vi "Build VIHelpeks Project.vi"(7 "Show Progress Window (T)":bool=TRUE, 8 "error in":errorcluster, 9 "Generate CHM (T)":bool=TRUE, 10 "Generate HHP (T)":bool=TRUE, 11 "VIHelpeks Project File":path) -> (0 "error out":errorcluster, 1 "Errors":i32, 2 "Paths":T1, 3 "dup VIHelpeks Project File":path)   [LabVIEW 2014, in "VIHelpeksAPI.lvlib"]
doc: "The VI builds help files based on a <b>VIHelpeks Project File</b>. The project file must be created and configured beforehand using the VI Helpeks UI (the help project manager). Information regarding the compiled project can be found in the files returned by the <b>Paths</b> indicator.\n\nThe VI generates a set of HTML files. In addition, if enabled, it generates project files for Microsoft HTML Help Workshop (.HHP and related files). Afterwards, if enabled, it compiles a final .CHM file based on the created (or already existing) .HHP and HTML files.\n\n<b>NOTICE:</b> In order to generate a CHM file, it is required to have Microsoft HTML Help Workshop installed on your computer. You can download it on the Microsoft website for free: <b>http://msdn.microsoft.com/en-us/library/ms669985.aspx</b>.\n\nThe <b>Example VI</b> demonstrating the use of VIHelpeks API can be opened using the \"Tools >> VI Helpeks >> Help and Support\" menu. Alternatively, you can launch the <b>NI Example Finder</b> and search for \"VI Helpeks\", or find it within the <b><labview>\\Examples\\VI Helpeks</b> folder.\n\n::: VI Helpeks :::\nCopyright (c) 2000-2026 Konstantin Shifershteyn. All rights reserved."
uses:
  VIHelpeksAPI.lvlib
  <vilib>/Utility/error.llb/DialogType.ctl
panel:
  in  "Show Window":bool
  out "VIHelpeks message":string
  # "VI Helpeks\nCopyright (c) 2012-2026 Konstantin Shifershteyn"
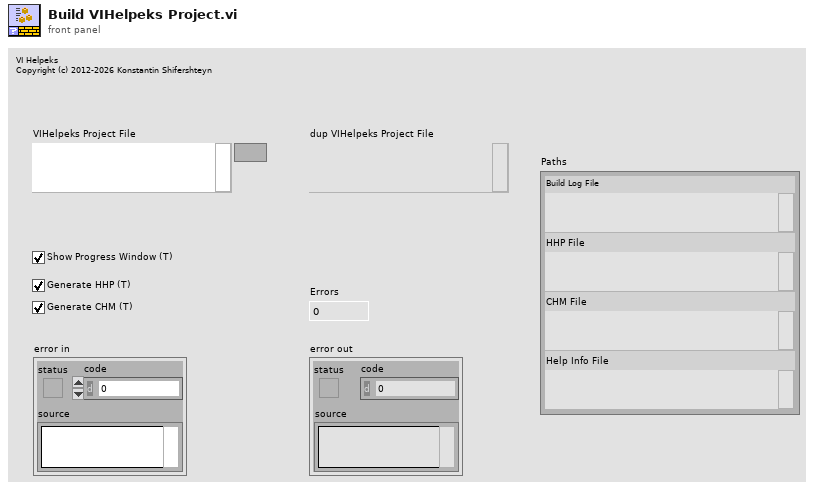
[diagram p1: front panel]
types:
  T1 = cluster{"Build Log File":path, "HHP File":path, "CHM File":path, "Help Info File":path}
  T2 = cluster{"HTML Build Log":path, "HHP File":path, "CHM File":path, "CHM Info File":path}
  T3 = cluster{"queue out":refnum<queue>, "queue out":refnum<queue>}
  T4 = cluster{"Msg":string, "Data":string, "error":errorcluster}
  T5 = enum32{"Bad", "Idle", "Run top level", "Running"}
  T6 = typedef "DialogType.ctl" = u16
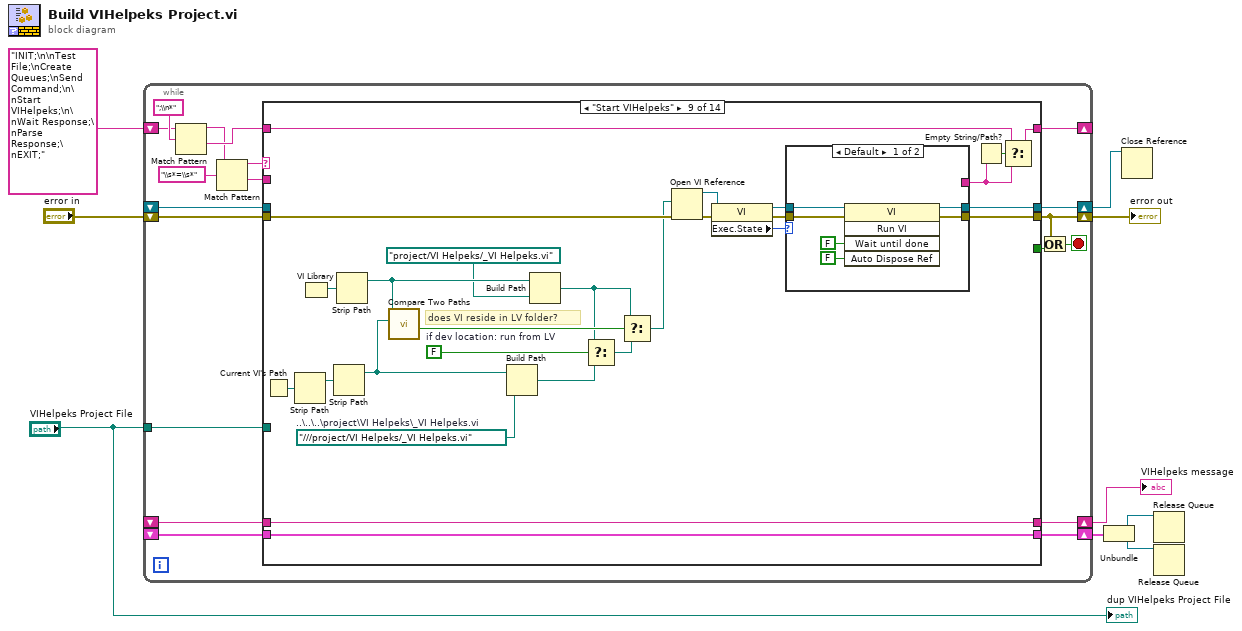
[diagram p0: block diagram]
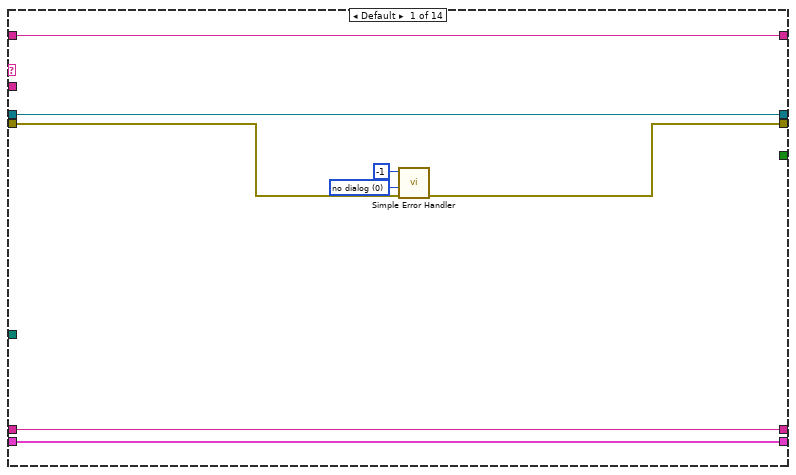
[diagram p2: hidden frame]
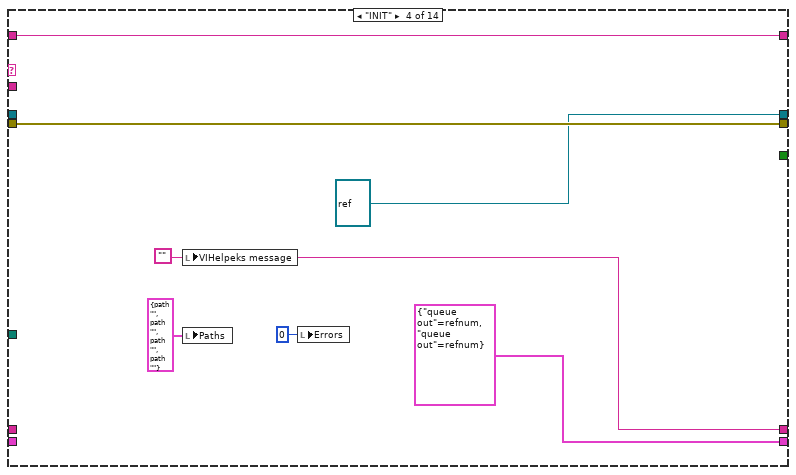
[diagram p5: hidden frame]
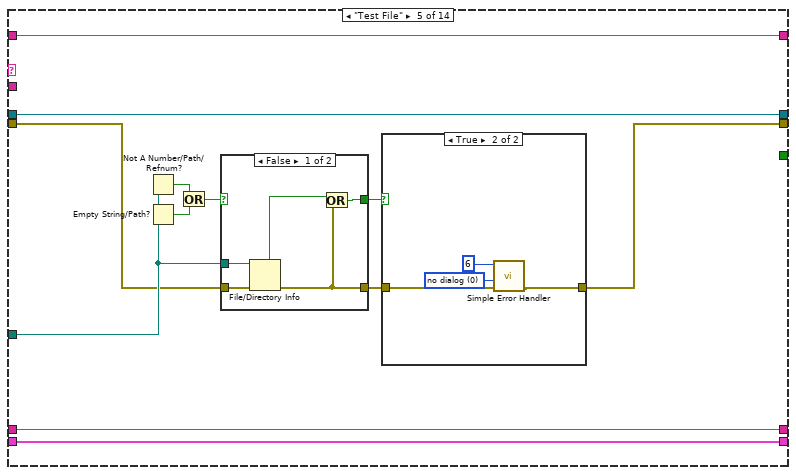
[diagram p6: hidden frame]
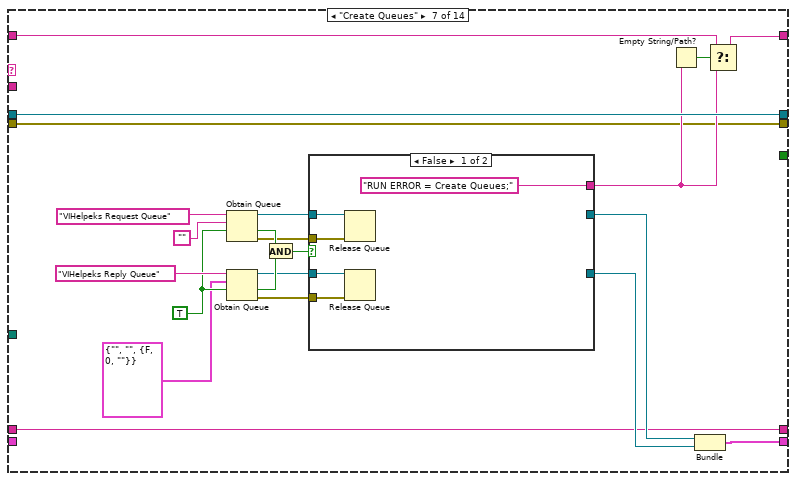
[diagram p10: hidden frame]
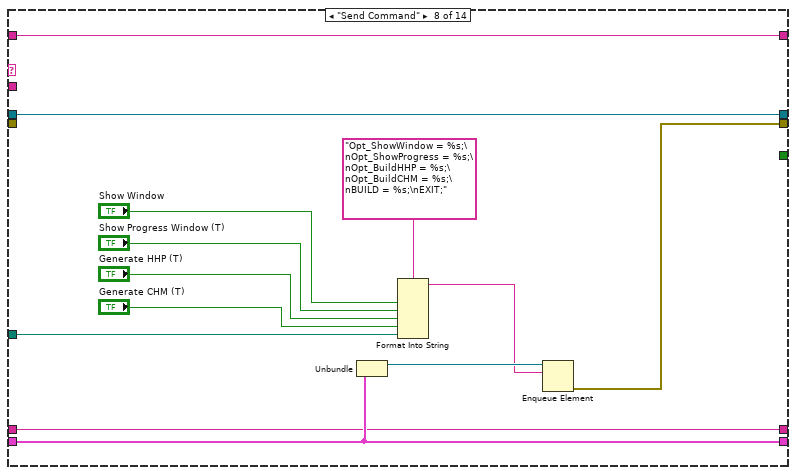
[diagram p12: hidden frame]
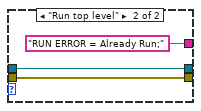
[diagram p13: hidden frame]
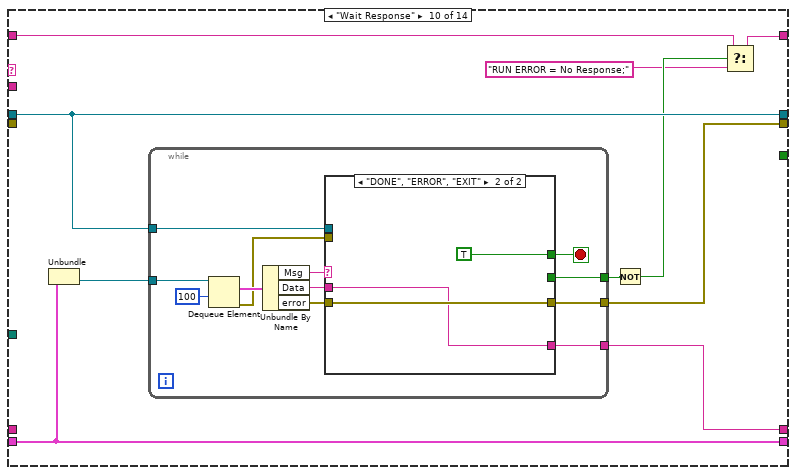
[diagram p14: hidden frame]
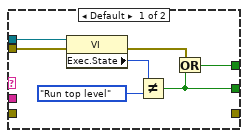
[diagram p15: hidden frame]
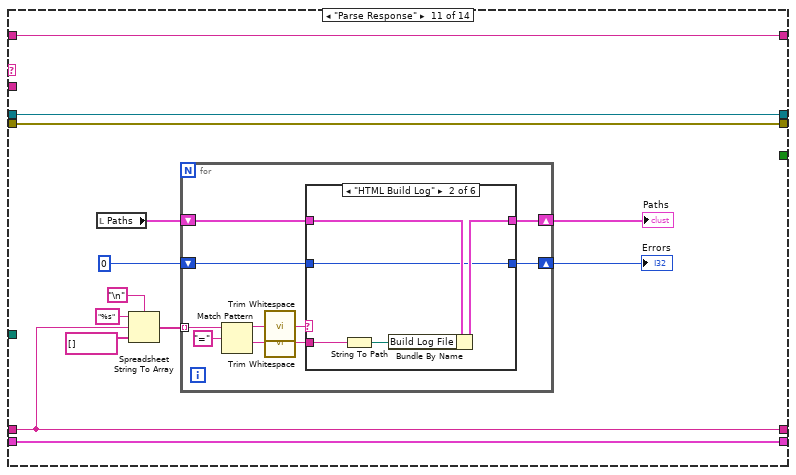
[diagram p16: hidden frame]
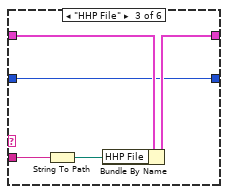
[diagram p18: hidden frame]
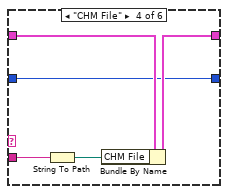
[diagram p19: hidden frame]
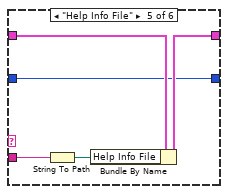
[diagram p20: hidden frame]
diagram:
  n1 = while {
    shift-right: [w26] -> _
    shift-left: "INIT;\n\nTest File;\nCreate Queues;\nSend Command;\n\nStart VIHelpeks;\n\nWait Response;\nParse Response;\nEXIT;" -> [w27]
    shift-right: [w19] -> w7
    shift-left: "error in" -> [w24]
    tunnel: "VIHelpeks Project File" -> [w22]
    shift-right: [w21] -> w6
    shift-left: _ -> [w20]
    shift-right: [w17] -> w5
    shift-left: _ -> [w16]
    shift-right: [w11] -> w2
    shift-left: _ -> [w10]
    stop <- w23 stop-if-true
    n2 = Match Pattern(string=w27, regular expression=";\\n*") -> (before substring=w15:string, after substring=w25:string)  [unwired: 1 in, 2 out]
    n3 = Match Pattern(string=w15, regular expression="\\s*=\\s*") -> (before substring=w13:string, after substring=w12:string)  [unwired: 1 in, 2 out]
    n4 = case shown="\"Start VIHelpeks\"" w13 {
      tunnel: [w36 w41 w46 w52 w57 w82 w87 w118 w140 w165 w205 w245 w262 w274] -> w26
      tunnel: w25 -> [w36 w41 w46 w52 w57 w82 w88 w118 w141 w161 w205 w245 w262 w274]
      tunnel: w24 -> [w35 w38 w43 w53 w60 w79 w84 _ w146 _ w203 w242 w258 w270]
      tunnel: [w34 w38 w43 w53 w59 w79 w84 w119 w145 w163 w203 w242 w257 w270] -> w19
      tunnel: w22 -> [_ _ _ _ w63 _ _ w121 _ _ _ _ _ _]
      tunnel: [w32 w40 w45 refnum<vi> refnum ("vi reference") w56 w81 w104 w124 w144 w168 w202 w244 w261 w273] -> w21
      tunnel: w20 -> [w32 w40 w45 _ w56 w81 w104 w124 _ w168 w202 w244 w261 w273]
      tunnel: [_ _ _ _ _ _ _ _ _ _ _ _ TRUE TRUE] -> w18
      tunnel: [w31 w39 w44 T3 {"queue out"=refnum, "queue out"=refnum} ("output cluster") w55 w80 w90 w123 w143 w170 w204 w243 w259 w271] -> w17
      tunnel: w16 -> [w31 w39 w44 _ w55 w80 _ w123 w143 w170 w204 w243 w259 w271]
      tunnel: w12 -> [_ _ _ _ _ _ _ _ _ _ _ _ w255 _]
      tunnel: [w29 w37 w42 w49 w54 w78 w83 w112 w128 w162 w200 w241 w246 w269] -> w11
      tunnel: w10 -> [w29 w37 w42 _ w54 w78 w83 w112 w128 _ w200 w241 w246 w269]
      frame Default {
        w30 = T6 0 items=["no dialog", "OK message", "continue or stop message", "OK message + warnings", "continue/stop + warnings"] ("type of dialog (OK msg:1)")
        n5 = call <vilib>:"Simple Error Handler.vi"("error code (no error:0)"=-1, "type of dialog (OK msg:1)"=w30, "error in (no error)"=w35) -> ("error out"=w34:errorcluster)  [unwired: 2 in, 4 out]
      }
      frame "" {
      }
      frame "------------------- 1" {
      }
      frame "INIT" {
        w49 = ""
        n6 = local write "VIHelpeks message"(w49) -> ()
        n7 = local write "Paths"(T2 {"HTML Build Log"=path "", "HHP File"=path "", "CHM File"=path "", "CHM Info File"=path ""} ("Paths")) -> ()
        n8 = local write "Errors"(0 ("Errors")) -> ()
      }
      frame "Test File" {
        n9 = Not A Number/Path/Refnum?(number/path/refnum=w63) -> (NaN/Path/Refnum?=w65:bool)
        n10 = Empty String/Path?(string/path=w63) -> (empty?=w64:bool)
        n11 = Or(x=w65, y=w64) -> (x .or. y?=w62:bool)
        n12 = case shown="False" w62 {
          selector: w62 -> [_ w77]
          tunnel: w63 -> [w75 _]
          tunnel: [w74 w77] -> w61
          tunnel: w60 -> [w72 w76]
          tunnel: [w71 w76] -> w58
          frame False {
            n13 = File/Directory Info(path=w75, error in=w72) -> (directory=w73:bool, error out=w71:errorcluster)  [unwired: 5 out]
            n14 = Or(x=w73, y=w71) -> (x .or. y?=w74:bool)
          }
          frame True {
          }
        }
        n15 = case shown="True" w61 {
          tunnel: [w66 w69] -> w59
          tunnel: w58 -> [w66 w70]
          frame False {
          }
          frame True {
            w67 = T6 0 items=["no dialog", "OK message", "continue or stop message", "OK message + warnings", "continue/stop + warnings"] ("type of dialog (OK msg:1)")
            n16 = call <vilib>:"Simple Error Handler.vi"("error code (no error:0)"=6, "type of dialog (OK msg:1)"=w67, "error in (no error)"=w70) -> ("error out"=w69:errorcluster)  [unwired: 2 in, 4 out]
          }
        }
      }
      frame "------------------- 2" {
      }
      frame "Create Queues" {
        w100 = TRUE
        n17 = Obtain Queue(name (unnamed)="VIHelpeks Request Queue", element data type="", create if not found? (T)=w100) -> (queue out=w96:refnum<queue>, created new?=w99:bool, error out=w94:errorcluster)  [unwired: 2 in]
        n18 = Obtain Queue(name (unnamed)="VIHelpeks Reply Queue", element data type=T4 {"Msg"="", "Data"="", "error"={"status"=FALSE, "code"=0, "source"=""}}, create if not found? (T)=w100) -> (queue out=w95:refnum<queue>, created new?=w98:bool, error out=w93:errorcluster)  [unwired: 2 in]
        n19 = And(x=w99, y=w98) -> (x .and. y?=w97:bool)
        n20 = case shown="False" w97 {
          tunnel: [_ w111] -> w92
          tunnel: w96 -> [w108 w111]
          tunnel: [_ w110] -> w91
          tunnel: w95 -> [w109 w110]
          tunnel: w94 -> [w107 _]
          tunnel: w93 -> [w106 _]
          tunnel: ["RUN ERROR = Create Queues;" _] -> w86
          frame False {
            n21 = Release Queue(queue=w108, error in (no error)=w107) -> ()  [unwired: 1 in, 3 out]
            n22 = Release Queue(queue=w109, error in (no error)=w106) -> ()  [unwired: 1 in, 3 out]
          }
          frame True {
          }
        }
        n23 = Empty String/Path?(string/path=w86) -> (empty?=w85:bool)
        n24 = Bundle("queue out"=w92, "queue out"=w91) -> (w90:T3)  [unwired: 1 in]
        n25 = Select(t=w88, s=w85, f=w86) -> (s? t:f=w87:string)
      }
      frame "Send Command" {
        n26 = Unbundle(w123) -> ("queue out"=w122:refnum<queue>)  [unwired: 1 out]
        n27 = Format Into String(format string="Opt_ShowWindow = %s;\nOpt_ShowProgress = %s;\nOpt_BuildHHP = %s;\nOpt_BuildCHM = %s;\nBUILD = %s;\nEXIT;", "Show Window", "Show Progress Window (T)", "Generate HHP (T)", "Generate CHM (T)", w121) -> (resulting string=w120:string)  [unwired: 2 in, 1 out]
        n28 = Enqueue Element(queue=w122, element=w120) -> (error out=w119:errorcluster)  [unwired: 2 in, 2 out]
      }
      frame "Start VIHelpeks" {
        w130 = FALSE  # if dev location: run from LV
        w134 = path "../../../project/VI Helpeks/_VI Helpeks.vi"  # ..\..\..\project\VI Helpeks\_VI Helpeks.vi
        # "does VI reside in LV folder?"
        n29 = Current VI's Path() -> (path=w127:path)
        n30 = Strip Path(path=w127) -> (stripped path=w126:path)  [unwired: 1 out]
        n31 = VI Library() -> (path=w138:path)
        n32 = Strip Path(path=w126) -> (stripped path=w125:path)  [unwired: 1 out]
        n33 = Strip Path(path=w138) -> (stripped path=w137:path)  [unwired: 1 out]
        n34 = call <vilib>:"Compare Two Paths.vi"("Path 2"=w125, "Path 1"=w137) -> ("Path 2 Relative to Path 1?"=w135:bool)  [unwired: 6 in, 3 out]
        n35 = Build Path(base path=w125, name or relative path=w134) -> (appended path=w131:path)
        n36 = Build Path(base path=w137, name or relative path=path "project/VI Helpeks/_VI Helpeks.vi") -> (appended path=w133:path)
        n37 = Select(t=w133, s=w130, f=w131) -> (s? t:f=w132:path)
        n38 = Select(t=w133, s=w135, f=w132) -> (s? t:f=w129:path)
        n39 = Open VI Reference(vi path=w129, error in (no error)=w146) -> (vi reference=w148:refnum<vi>, error out=w147:errorcluster)  [unwired: 4 in]
        n40 = property class="VI"(reference=w148, error in=w147) -> (reference out=w151:refnum<vi>, error out=w150:errorcluster, "Exec.State"=w149:T5)
        n41 = case shown="Default" w149 {
          tunnel: [w153 w160] -> w145
          tunnel: w150 -> [w155 w160]
          tunnel: w151 -> [w154 w159]
          tunnel: [w152 w159] -> w144
          tunnel: [_ "RUN ERROR = Already Run;"] -> w139
          frame Default {
            n42 = invoke class="VI" method="Run VI"(reference=w154, error in=w155, "Wait until done"=FALSE ("Wait Until Done"), "Auto Dispose Ref"=FALSE ("Auto Dispose Reference")) -> (reference out=w152:refnum<vi>, error out=w153:errorcluster)  [unwired: 1 in, 3 out]
          }
          frame "Run top level" {
          }
        }
        n43 = Empty String/Path?(string/path=w139) -> (empty?=w142:bool)
        n44 = Select(t=w141, s=w142, f=w139) -> (s? t:f=w140:string)
      }
      frame "Wait Response" {
        n45 = Unbundle(w170) -> ("queue out"=w169:refnum<queue>)  [unwired: 1 out]
        n46 = while {
          tunnel: w169 -> [w182]
          tunnel: w168 -> [w177]
          tunnel: [w173] -> w167
          tunnel: [w172] -> w163
          tunnel: [w171] -> w162
          stop <- w176 stop-if-true
          n47 = Dequeue Element(queue=w182, timeout in ms (-1)=100) -> (element=w180:T4, error out=w175:errorcluster)  [unwired: 1 in, 2 out]
          n48 = Unbundle By Name(w180) -> ("Msg"=w179:string, "Data"=w174:string, "error"=w178:errorcluster)
          n49 = case shown="\"DONE\", \"ERROR\", \"EXIT\"" w179 {
            tunnel: w178 -> [_ w191]
            tunnel: w177 -> [w186 _]
            tunnel: [w185 TRUE] -> w176
            tunnel: w175 -> [w184 _]
            tunnel: w174 -> [_ w190]
            tunnel: [w183 _] -> w173
            tunnel: [_ w191] -> w172
            tunnel: [_ w190] -> w171
            frame Default {
              n50 = property class="VI"(reference=w186, error in=w184) -> (error out=w187:errorcluster, "Exec.State"=w189:T5)  [unwired: 1 out]
              n51 = Not Equal?(x=w189, y=T5."Run top level") -> (x != y?=w183:bool)
              n52 = Or(x=w187, y=w183) -> (x .or. y?=w185:bool)
            }
            frame "DONE", "ERROR", "EXIT" {
            }
          }
        }
        n53 = Not(x=w167) -> (.not. x?=w166:bool)
        n54 = Select(t=w161, s=w166, f="RUN ERROR = No Response;") -> (s? t:f=w165:string)
      }
      frame "Parse Response" {
        n55 = local read "Paths"() -> (w196:T1)
        n56 = Spreadsheet String To Array(delimiter (Tab)="\n", format string="%s", spreadsheet string=w200, array type (2D Dbl)=string[] []) -> (array=w197:string[])
        n57 = for {
          tunnel: w197 -> [w215] mode=indexing
          shift-right: [w210] -> w195
          shift-left: w196 -> [w209]
          shift-right: [w207] -> w194
          shift-left: 0 -> [w206]
          n58 = Match Pattern(string=w215, regular expression="=") -> (before substring=w213:string, after substring=w212:string)  [unwired: 1 in, 2 out]
          n59 = call <vilib>:"Trim Whitespace.vi"("string"=w213) -> ("trimmed string"=w211:string)  [unwired: 1 in]
          n60 = call <vilib>:"Trim Whitespace.vi"("string"=w212) -> ("trimmed string"=w208:string)  [unwired: 1 in]
          n61 = case shown="\"HTML Build Log\"" w211 {
            tunnel: [w217 w221 w226 w231 w236 w240] -> w210
            tunnel: w209 -> [w217 w222 w227 w232 w237 w240]
            tunnel: w208 -> [_ w220 w225 w230 w235 w239]
            tunnel: [w216 w218 w223 w228 w233 w238] -> w207
            tunnel: w206 -> [w216 w218 w223 w228 w233 _]
            frame Default {
            }
            frame "HTML Build Log" {
              n62 = String To Path(string=w220) -> (path=w219:path)
              n63 = Bundle By Name(cluster=w222, "Build Log File"=w219) -> (w221:T1)
            }
            frame "HHP File" {
              n64 = String To Path(string=w225) -> (path=w224:path)
              n65 = Bundle By Name(cluster=w227, "HHP File"=w224) -> (w226:T1)
            }
            frame "CHM File" {
              n66 = String To Path(string=w230) -> (path=w229:path)
              n67 = Bundle By Name(cluster=w232, "CHM File"=w229) -> (w231:T1)
            }
            frame "Help Info File" {
              n68 = String To Path(string=w235) -> (path=w234:path)
              n69 = Bundle By Name(cluster=w237, "Help Info File"=w234) -> (w236:T1)
            }
            frame "Num Of Errors" {
              n70 = Decimal String To Number(string=w239) -> (number=w238:i32)  [unwired: 2 in, 1 out]
            }
          }
        }
        "Paths" <- w195
        "Errors" <- w194
      }
      frame "------------------- 3" {
      }
      frame "RUN ERROR" {
        w256 = T6 0 items=["no dialog", "OK message", "continue or stop message", "OK message + warnings", "continue/stop + warnings"] ("type of dialog (OK msg:1)")
        n71 = case shown="\"Create Queues\"" w255 {
          tunnel: [_ "Error of starting VI Helpeks. It could be already running." "Error of starting VI Helpeks. It is already running." "VIHelpeks terminated without response. No build status is available."] -> w250
          tunnel: [_ 510100 510101 510102] -> w254
          frame Default {
          }
          frame "Create Queues" {
          }
          frame "Already Run" {
          }
          frame "No Response" {
          }
        }
        n72 = Call Chain() -> (call chain=w253:string[])
        n73 = Array To Spreadsheet String(delimiter (Tab)=" in ", array=w253, 3:"\"%s\"" ("format string")) -> (spreadsheet string=w249:string)
        n74 = Format Into String(format string="<ERR>%s", initial string=w249, w250) -> (resulting string=w248:string)  [unwired: 1 in, 1 out]
        n75 = call <vilib>:"Simple Error Handler.vi"("error code (no error:0)"=w254, "error source (\" \")"=w248, "type of dialog (OK msg:1)"=w256, "error in (no error)"=w258) -> ("error out"=w257:errorcluster)  [unwired: 1 in, 4 out]
      }
      frame "EXIT" {
      }
    }
    n76 = Or(x=w19, y=w18) -> (x .or. y?=w23:bool)
  }
  "error out" <- w7
  "VIHelpeks message" <- w2
  n77 = Unbundle(w5) -> ("queue out"=w4:refnum<queue>, "queue out"=w3:refnum<queue>)
  n78 = Close Reference(reference=w6) -> ()  [unwired: 1 in, 1 out]
  n79 = Release Queue(queue=w4) -> ()  [unwired: 2 in, 3 out]
  n80 = Release Queue(queue=w3) -> ()  [unwired: 2 in, 3 out]
  "dup VIHelpeks Project File" <- "VIHelpeks Project File"
